vi "Cut Curve.vi"(9 "X2":dbl format="%#_13g", 10 "X1":dbl format="%#_13g", 11 "Curve":cluster{"X":dbl[], "Y":dbl[]}={"X"=array[4260 elements], "Y"=array[4260 elements]}) -> (3 "Cut Curve":cluster{dbl[], dbl[]})   [LabVIEW 2020, in "Data Viewer.lvlib" / "Data Viewer.lvclass"]
uses:
  Data Viewer.lvclass
panel:
  in  "因子":dbl=1.0 format="%#_13g"
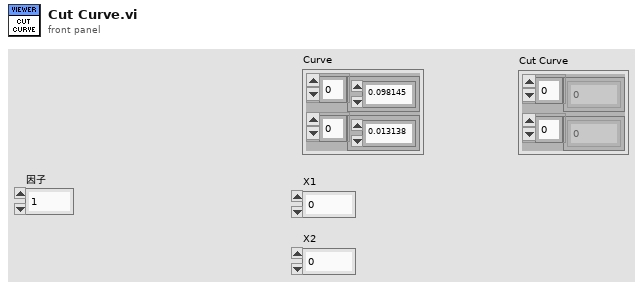
[diagram p1: front panel]
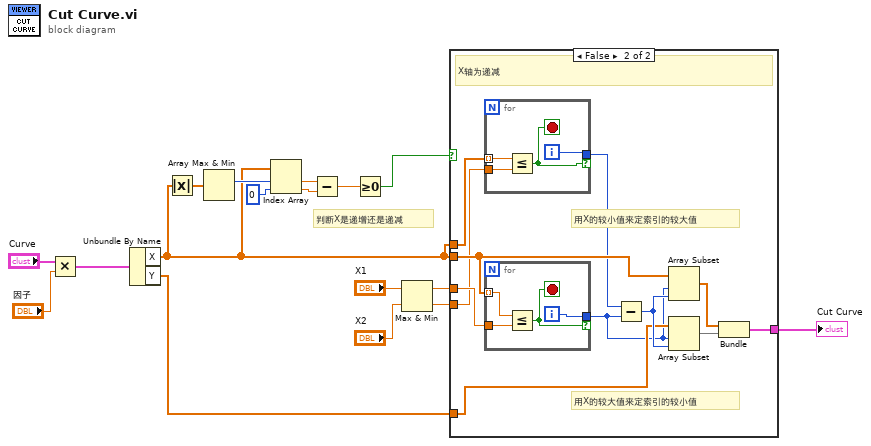
[diagram p0: block diagram]
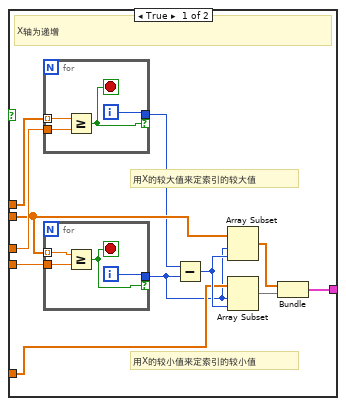
[diagram p2: hidden frame]
diagram:
  # "判断X是递增还是递减"
  n1 = Multiply(x="Curve", y="因子") -> (x*y=w14:cluster{"X":dbl[], "Y":dbl[]})
  n2 = Unbundle By Name(w14) -> ("X"=w4:dbl[], "Y"=w2:dbl[])
  n3 = Absolute Value(x=w4) -> (abs(x)=w12:dbl[])
  n4 = Array Max & Min(array=w12) -> (max index (indices)=w11:i32)  [unwired: 3 out]
  n5 = Index Array(array=w4, index #1=w11, index #2=0 ("索引")) -> (element #1=w8:dbl, element #2=w9:dbl)
  n6 = Subtract(x=w8, y=w9) -> (x-y=w7:dbl)
  n7 = Greater Or Equal To 0?(x=w7) -> (x >= 0?=w6:bool)
  n8 = Max & Min(x="X1", y="X2") -> (max(x,y)=w3:dbl, min(x,y)=w5:dbl)
  n9 = case shown="False" w6 {
    tunnel: w5 -> [w28 w37]
    tunnel: w4 -> [w24 w45]
    tunnel: w4 -> [w27 w47]
    tunnel: w3 -> [w26 w38]
    tunnel: w2 -> [w23 w44]
    tunnel: [w20 w41] -> w1
    frame True {
      # "用X的较大值来定索引的较大值"
      # "用X的较小值来定索引的较小值"
      # "X轴为递增"
      n10 = for {
        tunnel: w27 -> [w31] mode=indexing
        tunnel: w26 -> [w32]
        tunnel: [w30] -> w19 if=w29
        i -> [w30]
        stop <- w29 stop-if-true
        n11 = Greater Or Equal?(x=w31, y=w32) -> (x >= y?=w29:bool)
      }
      n12 = for {
        tunnel: w24 -> [w35] mode=indexing
        tunnel: w28 -> [w36]
        tunnel: [w34] -> w18 if=w33
        i -> [w34]
        stop <- w33 stop-if-true
        n13 = Greater Or Equal?(x=w35, y=w36) -> (x >= y?=w33:bool)
      }
      n14 = Subtract(x=w19, y=w18) -> (x-y=w25:i32)
      n15 = Array Subset(array=w24, index=w18, length=w25) -> (w22:dbl[])
      n16 = Array Subset(array=w23, index=w18, length=w25) -> (w21:dbl[])
      n17 = Bundle(w22, w21) -> (w20:cluster{dbl[], dbl[]})  [unwired: 1 in]
    }
    frame False {
      # "用X的较小值来定索引的较大值"
      # "用X的较大值来定索引的较小值"
      # "X轴为递减"
      n18 = for {
        tunnel: w47 -> [w50] mode=indexing
        tunnel: w37 -> [w51]
        tunnel: [w49] -> w40 if=w48
        i -> [w49]
        stop <- w48 stop-if-true
        n19 = Less Or Equal?(x=w50, y=w51) -> (x <= y?=w48:bool)
      }
      n20 = for {
        tunnel: w45 -> [w54] mode=indexing
        tunnel: w38 -> [w55]
        tunnel: [w53] -> w39 if=w52
        i -> [w53]
        stop <- w52 stop-if-true
        n21 = Less Or Equal?(x=w54, y=w55) -> (x <= y?=w52:bool)
      }
      n22 = Subtract(x=w40, y=w39) -> (x-y=w46:i32)
      n23 = Array Subset(array=w45, index=w39, length=w46) -> (w43:dbl[])
      n24 = Array Subset(array=w44, index=w39, length=w46) -> (w42:dbl[])
      n25 = Bundle(w43, w42) -> (w41:cluster{dbl[], dbl[]})  [unwired: 1 in]
    }
  }
  "Cut Curve" <- w1
